vi "WordsToI32(SubVI).vi"(0 "배열":u16[][](array[numeric]), 5 "인덱스 (열)":i32, 7 "인덱스":i32, 9 "길이":i32, 11 "error input":errorcluster) -> (4 "array output":i32[](array[numeric]), 15 "error out":errorcluster)   [LabVIEW 2019]
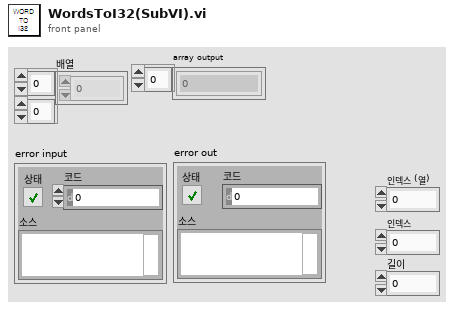
[diagram p1: front panel]
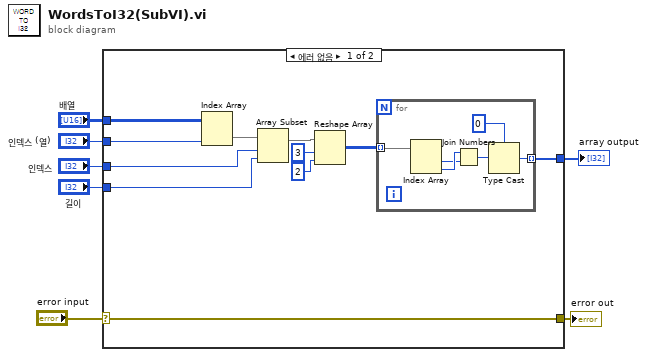
[diagram p0: block diagram]
diagram:
  n1 = case shown="에러 없음" "error input" {
    selector: "error input" -> [w15 w25]
    tunnel: [w15 w25] -> w6
    tunnel: "배열" -> [w14 _]
    tunnel: [w11 _] -> w5
    tunnel: "인덱스 (열)" -> [w10 _]
    tunnel: "길이" -> [w9 _]
    tunnel: "인덱스" -> [w8 _]
    frame No Error {
      n2 = Index Array(array=w14, index (col)=w10) -> (element=w12:u16[])  [unwired: 1 in]
      n3 = Array Subset(array=w12, index=w8, length=w9) -> (w13:u16[])
      n4 = Reshape Array(w13, 3 ("차원 크기"), 2 ("차원 크기")) -> (w16:u16[][])
      n5 = for {
        tunnel: w16 -> [w24] mode=indexing
        tunnel: [w21] -> w11 mode=indexing
        n6 = Index Array(array=w24) -> (element #1=w19:u16, element #2=w20:u16)  [unwired: 2 in]
        n7 = Join Numbers(hi=w20, lo=w19) -> ((hi.lo)=w23:u32)
        n8 = Type Cast(type=0, x=w23) -> (*(type *) &x=w21:i32)
      }
    }
    frame Error {
    }
  }
  "error out" <- w6
  "array output" <- w5
